vi "AI_Calculate_Move.vi"(0 "Grid":enum8{"Empty", "Black", "White"}[][](array[ring])=[[enum."Empty", enum."Empty", enum."Empty", enum."Empty", enum."Empty", enum."Empty", enum."Empty", enum."Empty", enum."Empty", enum."Empty", enum."Empty", enum."Empty", enum."Empty", enum."Empty", enum."Empty"], [enum."Empty", enum."Empty", enum."Empty", enum."Empty", enum."Empty", enum."Empty", enum."Empty", enum."Empty", enum."Empty", enum."Empty", enum."Empty", enum."Empty", enum."Empty", enum."Empty", enum."Empty"], [enum."Empty", enum."Empty", enum."Empty", enum."Empty", enum."Empty", enum."Empty", enum."Empty", enum."Empty", enum."Empty", enum."Empty", enum."Empty", enum."Empty", enum."Empty", enum."Empty", enum."Empty"], [enum."Empty", enum."Empty", enum."Empty", enum."Empty", enum."Empty", enum."Empty", enum."Empty", enum."Empty", enum."Empty", enum."Empty", enum."Empty", enum."Empty", enum."Empty", enum."Empty", enum."Empty"], [enum."Empty", enum."Empty", enum."Empty", enum."Empty", enum."Empty", enum."Empty", enum."Empty", enum."Empty", enum."Empty", enum."Empty", enum."Empty", enum."Empty", enum."Empty", enum."Empty", enum."Empty"], [enum."Empty", enum."Empty", enum."Empty", enum."Empty", enum."Empty", enum."Empty", enum."Empty", enum."Empty", enum."Empty", enum."Empty", enum."Empty", enum."Empty", enum."Empty", enum."Empty", enum."Empty"], [enum."Empty", enum."Empty", enum."Empty", enum."Empty", enum."Empty", enum."Empty", enum."Empty", enum."Empty", enum."Empty", enum."Empty", enum."Empty", enum."Empty", enum."Empty", enum."Empty", enum."Empty"], [enum."Empty", enum."Empty", enum."Empty", enum."Empty", enum."Empty", enum."Empty", enum."Empty", enum."Empty", enum."Empty", enum."Empty", enum."Empty", enum."Empty", enum."Empty", enum."Empty", enum."Empty"], [enum."Empty", enum."Empty", enum."Empty", enum."Empty", enum."Empty", enum."Empty", enum."Empty", enum."Empty", enum."Empty", enum."Empty", enum."Empty", enum."Empty", enum."Empty", enum."Empty", enum."Empty"], [enum."Empty", enum."Empty", enum."Empty", enum."Empty", enum."Empty", enum."Empty", enum."Empty", enum."Empty", enum."Empty", enum."Empty", enum."Empty", enum."Empty", enum."Empty", enum."Empty", enum."Empty"], [enum."Empty", enum."Empty", enum."Empty", enum."Empty", enum."Empty", enum."Empty", enum."Empty", enum."Empty", enum."Empty", enum."Empty", enum."Empty", enum."Empty", enum."Empty", enum."Empty", enum."Empty"], [enum."Empty", enum."Empty", enum."Empty", enum."Empty", enum."Empty", enum."Empty", enum."Empty", enum."Empty", enum."Empty", enum."Empty", enum."Empty", enum."Empty", enum."Empty", enum."Empty", enum."Empty"], [enum."Empty", enum."Empty", enum."Empty", enum."Empty", enum."Empty", enum."Empty", enum."Empty", enum."Empty", enum."Empty", enum."Empty", enum."Empty", enum."Empty", enum."Empty", enum."Empty", enum."Empty"], [enum."Empty", enum."Empty", enum."Empty", enum."Empty", enum."Empty", enum."Empty", enum."Empty", enum."Empty", enum."Empty", enum."Empty", enum."Empty", enum."Empty", enum."Empty", enum."Empty", enum."Empty"], [enum."Empty", enum."Empty", enum."Empty", enum."Empty", enum."Empty", enum."Empty", enum."Empty", enum."Empty", enum."Empty", enum."Empty", enum."Empty", enum."Empty", enum."Empty", enum."Empty", enum."Empty"]], 5 "AI Stone":enum8{"Empty", "Black", "White"}(ring)=enum."White", 7 "Difficulty":enum8{"Easy", "Normal", "Hard", "Master"}(ring)=enum."Normal", 9 "Renju":bool=TRUE, 11 "error in":errorcluster) -> (4 "Move":T1={"Row"=-1, "Col"=-1, "Stone"=enum."Empty"}, 6 "Score":dbl, 8 "Valid":bool, 15 "error out":errorcluster)   [LabVIEW 2026]
doc: "AI 착수 결정. Easy=탐욕+큰 잡음, Normal=탐욕(공격+0.9*수비), Hard=상위 6후보, Master=상위 12후보에 상대 최선 응수를 빼는 2수 탐색.\nValid=False면 둘 곳이 없음(무승부)."
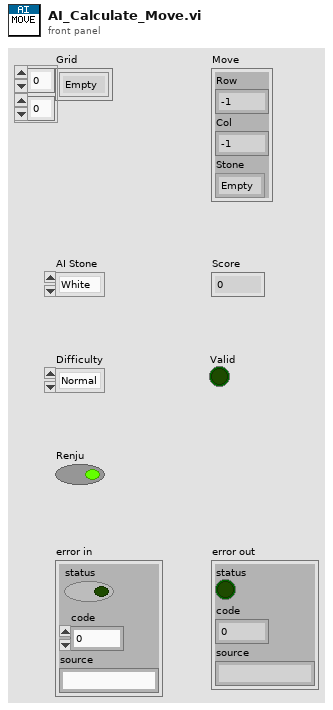
[diagram p1: front panel]
types:
  T1 = cluster{"Row":i32, "Col":i32, "Stone":enum8{"Empty", "Black", "White"}}
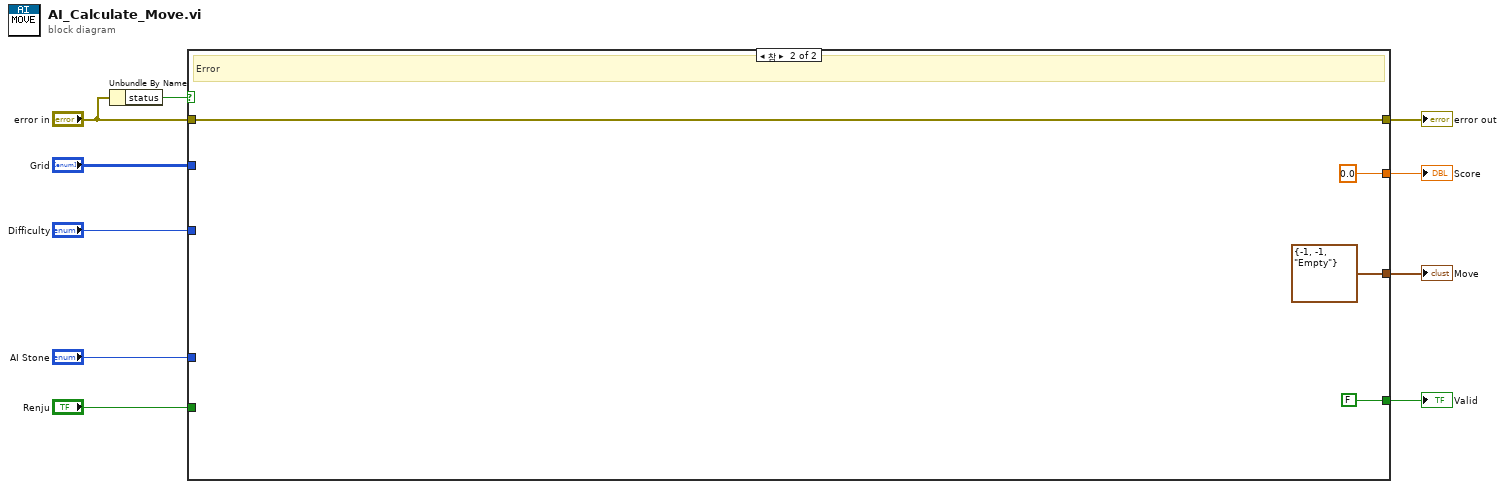
[diagram p0: block diagram]
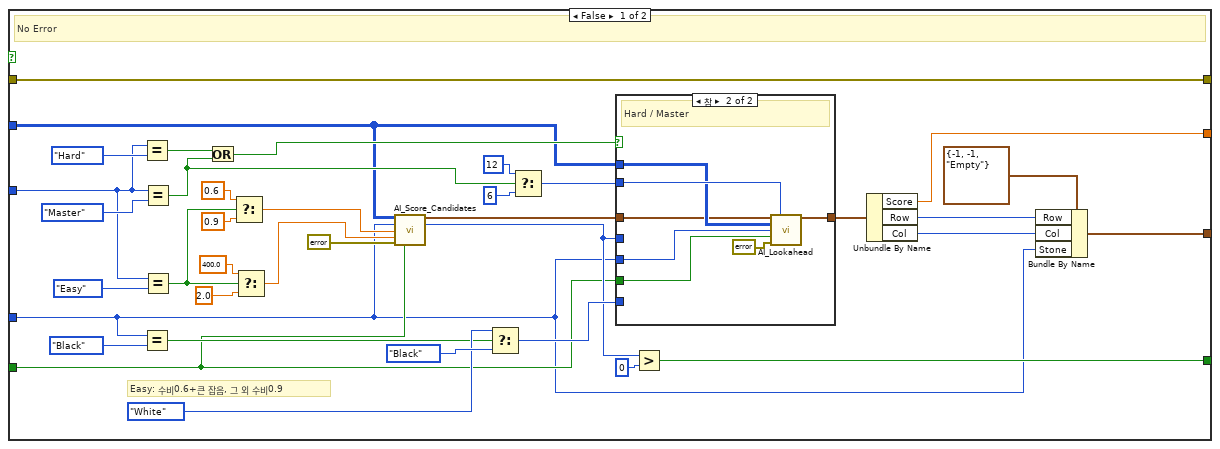
[diagram p2: hidden frame]
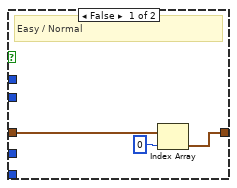
[diagram p3: hidden frame]
diagram:
  n1 = Unbundle By Name("error in") -> ("status"=w6:bool)
  n2 = case shown="참" w6 {
    tunnel: "Grid" -> [w11 _]
    tunnel: "AI Stone" -> [w12 _]
    tunnel: "Difficulty" -> [w13 _]
    tunnel: "Renju" -> [w14 _]
    tunnel: "error in" -> [w15 w58]
    tunnel: [w15 w58] -> w10
    tunnel: [w47 FALSE] -> w9
    tunnel: [w41 0.0] -> w8
    tunnel: [w45 T1 {"Row"=-1, "Col"=-1, "Stone"=enum."Empty"}] -> w7
    frame False {
      # "Easy: 수비0.6+큰 잡음, 그 외 수비0.9"
      # "No Error"
      n3 = Equal?(x=w13, y=enum8{"Easy", "Normal", "Hard", "Master"}."Hard") -> (x = y?=w21:bool)
      n4 = Equal?(x=w12, y=enum8{"Empty", "Black", "White"}."Black") -> (x = y?=w36:bool)
      n5 = Equal?(x=w13, y=enum8{"Easy", "Normal", "Hard", "Master"}."Master") -> (x = y?=w19:bool)
      n6 = Equal?(x=w13, y=enum8{"Easy", "Normal", "Hard", "Master"}."Easy") -> (x = y?=w17:bool)
      n7 = Or(x=w21, y=w19) -> (x .or. y?=w22:bool)
      n8 = Select(t=0.6, s=w17, f=0.9) -> (s? t:f=w28:dbl)
      n9 = Select(t=400.0, s=w17, f=2.0) -> (s? t:f=w31:dbl)
      n10 = call "AI_Score_Candidates.vi"("Grid"=w11, "AI Stone"=w12, "Defense Weight"=w28, "Noise"=w31, "error in"=errorcluster {"status"=FALSE, "code"=0, "source"=""}, "Renju"=w14) -> ("Ranked"=w33:cluster{"Score":dbl, "Row":i32, "Col":i32}[], "Count"=w34:i32)  [unwired: 7 in, 1 out]
      n11 = Select(t=enum8{"Empty", "Black", "White"}."White", s=w36, f=enum8{"Empty", "Black", "White"}."Black") -> (s? t:f=w39:enum8{"Empty", "Black", "White"})
      n12 = Select(t=12, s=w19, f=6) -> (s? t:f=w25:i32)
      n13 = case shown="참" w22 {
        tunnel: w11 -> [_ w52]
        tunnel: w12 -> [_ w53]
        tunnel: w14 -> [_ w54]
        tunnel: w39 -> [_ _]
        tunnel: w25 -> [_ w55]
        tunnel: w33 -> [w48 w51]
        tunnel: w34 -> [_ _]
        tunnel: [w50 w57] -> w40
        frame False {
          # "Easy / Normal"
          n14 = Index Array(array=w48, index=0) -> (element=w50:cluster{"Score":dbl, "Row":i32, "Col":i32})
        }
        frame True {
          # "Hard / Master"
          n15 = call "AI_Lookahead.vi"("Ranked"=w51, "Top K"=w55, "Grid"=w52, "AI Stone"=w53, "Renju"=w54, "error in"=errorcluster {"status"=FALSE, "code"=0, "source"=""}) -> ("Best"=w57:cluster{"Score":dbl, "Row":i32, "Col":i32})  [unwired: 7 in, 2 out]
        }
      }
      n16 = Greater?(x=w34, y=0) -> (0:w47:bool)
      n17 = Unbundle By Name(w40) -> ("Score"=w41:dbl, "Row"=w42:i32, "Col"=w43:i32)
      n18 = Bundle By Name(cluster=T1 {"Row"=-1, "Col"=-1, "Stone"=enum."Empty"}, "Row"=w42, "Col"=w43, "Stone"=w12) -> (w45:T1)
    }
    frame True {
      # "Error"
    }
  }
  "Move" <- w7
  "Score" <- w8
  "Valid" <- w9
  "error out" <- w10
